vi "server_subfolder_search.vi"(7 "SHz_selection":enum16{"10k", "100k"}(ring), 8 "error in":errorcluster, 9 "selection":u16(ring) items=["HU"], 10 "1folder names":string[](array[string]), 11 "present_s_path":path) -> (0 "error out":errorcluster, 1 "FOL#":i32, 2 "F_array_Link":path[](array[path]), 3 "Folder_List":string[](array[string]), 4 "element":string, 5 "2folder_name":string[](array[string]))   [LabVIEW 2018]
panel:
  out "1st":path[](array[path])
  out "2nd":path[](array[path])
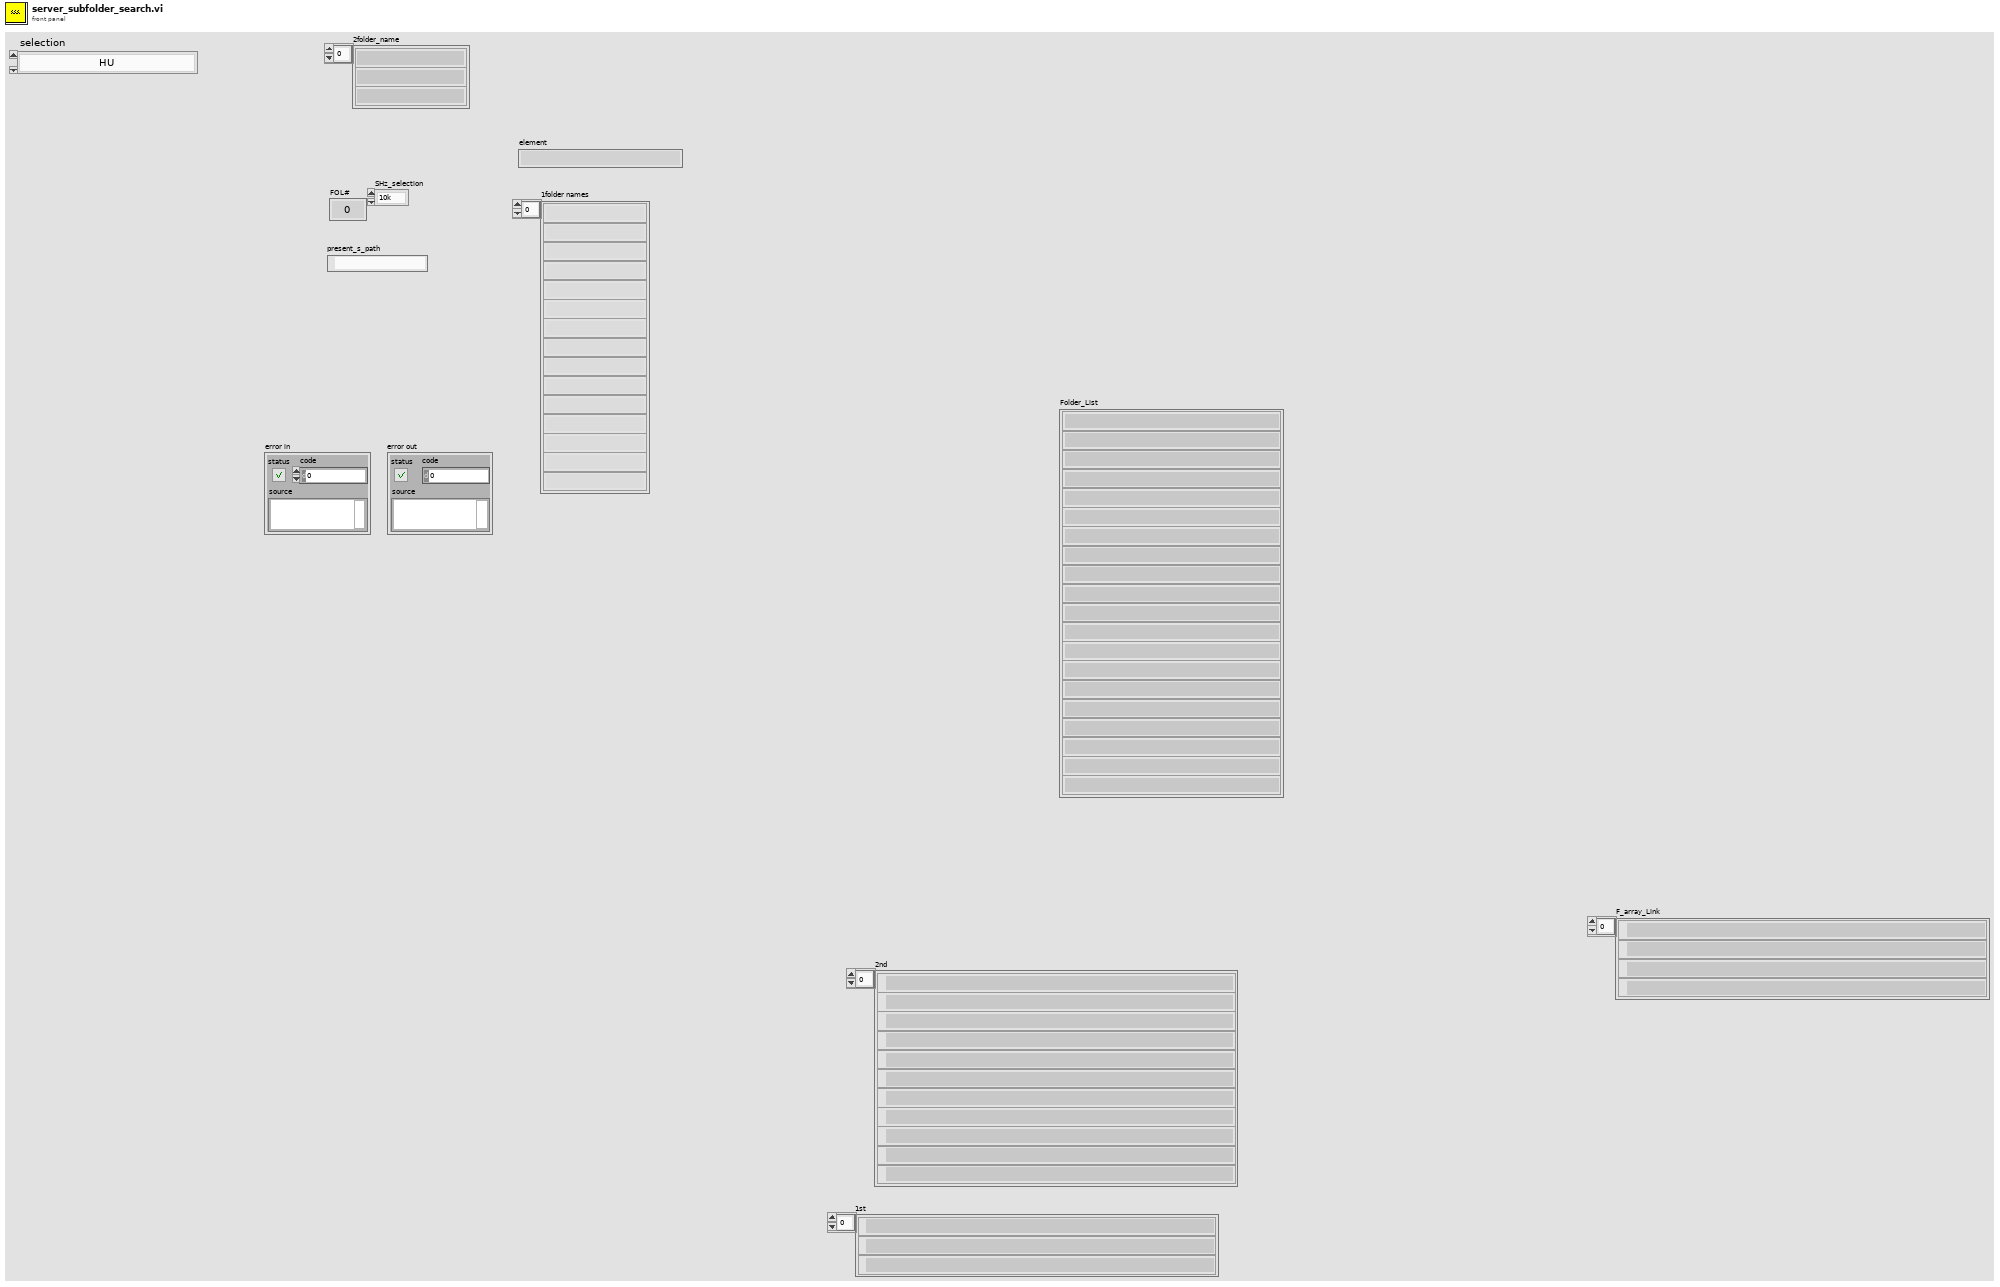
[diagram p1: front panel]
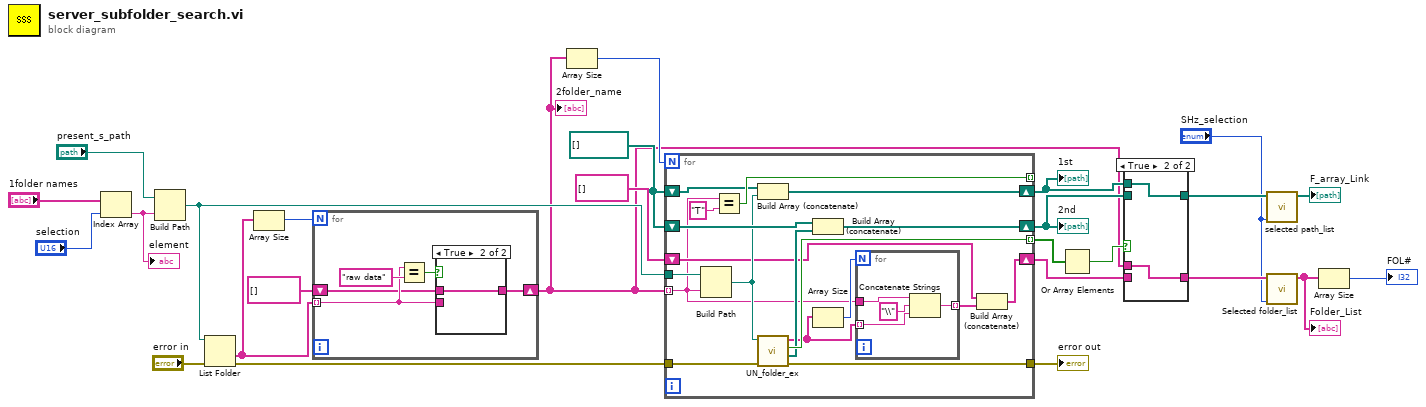
[diagram p0: block diagram]
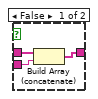
[diagram p3: hidden frame]
diagram:
  w17 = path[] []
  n1 = Index Array(array="1folder names", index="selection") -> (element=w5:string)
  "element" <- w5
  n2 = Build Path(base path="present_s_path", name or relative path=w5) -> (appended path=w15:path)
  n3 = List Folder(path=w15, error in="error in") -> (folder names=w23:string[], error out=w3:errorcluster)  [unwired: 2 in, 2 out]
  n4 = Array Size(array=w23) -> (size(s)=w24:i32)
  n5 = for {
    N: w24 -> [_]
    tunnel: w23 -> [w29] mode=indexing
    shift-right: [w28] -> w9
    shift-left: string[] [] -> [w27]
    n6 = Equal?(x=w29, y="raw data") -> (x = y?=w30:bool)
    n7 = case shown="True" w30 {
      tunnel: w29 -> [w34 _]
      tunnel: [w33 w35] -> w28
      tunnel: w27 -> [w32 w35]
      frame False {
        n8 = Build Array (concatenate)(w32, w34) -> (w33:string[])
      }
      frame True {
      }
    }
  }
  "2folder_name" <- w9
  n9 = Array Size(array=w9) -> (size(s)=w26:i32)
  n10 = for {
    N: w26 -> [_]
    tunnel: w9 -> [w39] mode=indexing
    tunnel: [w52] -> _ mode=indexing
    tunnel: w15 -> [w51]
    tunnel: [w50] -> w2
    tunnel: [w49] -> w25 mode=indexing
    shift-right: [w47] -> w21
    shift-left: w17 -> [w46]
    shift-right: [w44] -> w20
    shift-left: w17 -> [w43]
    shift-right: [w42] -> w19
    shift-left: string[] [] -> [w41]
    tunnel: w3 -> [w36]
    n11 = Build Path(base path=w51, name or relative path=w39) -> (appended path=w45:path)
    n12 = Equal?(x=w39, y="T" ("regular expression")) -> (x = y?=w52:bool)
    n13 = Build Array (concatenate)(w43, w45) -> (w44:path[])
    n14 = call "UN_folder_ex.vi"("error in"=w36, "path"=w45) -> ("error out"=w50:errorcluster, "Array"=w48:path[], "logical OR"=w49:bool, "foldername"=w38:string[])  [unwired: 6 in]
    n15 = Build Array (concatenate)(w46, w48) -> (w47:path[])
    n16 = Array Size(array=w38) -> (size(s)=w40:i32)
    n17 = for {
      N: w40 -> [_]
      tunnel: w39 -> [w57]
      tunnel: w38 -> [w56] mode=indexing
      tunnel: [w54] -> w37 mode=indexing
      n18 = Concatenate Strings(w57, "\\" ("string"), w56) -> (w54:string)
    }
    n19 = Build Array (concatenate)(w41, w37) -> (w42:string[])
  }
  "2nd" <- w21
  "1st" <- w20
  "error out" <- w2
  n20 = Or Array Elements(Boolean array=w25) -> (logical OR=w22:bool)
  n21 = case shown="True" w22 {
    tunnel: w21 -> [w59 _]
    tunnel: [w59 w61] -> w14
    tunnel: w20 -> [_ w61]
    tunnel: w9 -> [_ w60]
    tunnel: w19 -> [w58 _]
    tunnel: [w58 w60] -> w13
    frame False {
    }
    frame True {
    }
  }
  n22 = call "selected path_list.vi"("selection"="SHz_selection", "F_array_Link"=w14) -> ("Selected F_array_Link"=→"F_array_Link":path[])  [unwired: 9 in]
  n23 = call "Selected folder_list.vi"("selection"="SHz_selection", "Folder_List"=w13) -> ("selected Folder List"=w10:string[])  [unwired: 9 in]
  "Folder_List" <- w10
  n24 = Array Size(array=w10) -> (size(s)=→"FOL#":i32)
